vi "GetCursorPos Wrapper Template.vi"(11 "error in":errorcluster) -> (4 "X":i32, 6 "Y":i32, 8 "return value":i32, 15 "error out":errorcluster)   [LabVIEW 2020]
doc: "Reads the mouse cursor position in SCREEN coordinates through user32.dll GetCursorPos (stdcall, called in any thread). The point travels to the DLL as a POINT {LONG x, LONG y} that the function overwrites in place. return value is the Win32 BOOL: non-zero on success, 0 on failure. When error in carries an error the DLL is not called. Generated by tools\\Build Win32 Wrappers.vi - do not edit by hand, rebuild it."
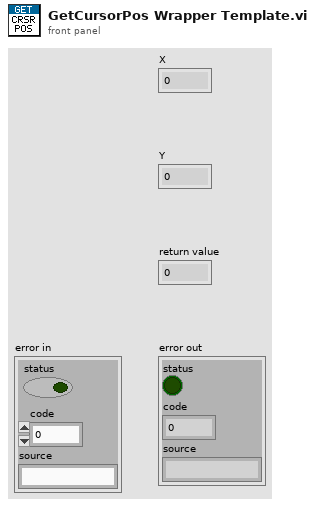
[diagram p1: front panel]
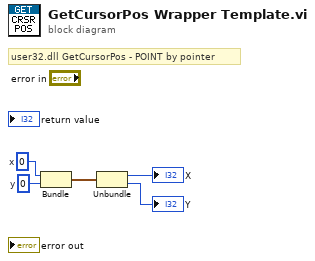
[diagram p0: block diagram]
diagram:
  w4 = 0  # y
  w3 = 0  # x
  # "user32.dll GetCursorPos - POINT by pointer"
  n1 = Bundle("x"=w3, "y"=w4) -> (w5:cluster{"x":i32, "y":i32})  [unwired: 1 in]
  n2 = Unbundle(w5) -> ("x"=→"X":i32, "y"=→"Y":i32)
